vi "VHist - Time Range from history array.vi"(1 "history array":T1(array[cluster]) {"history data" format="%.2f"; "time stamps" format="%<%H:%M:%S%2u\n%d/%m/%Y>T"}) -> (4 "max time stamp":dbl format="%<%H:%M:%S%2u\n%d/%m/%Y>T", 5 "min time stamp":dbl format="%<%H:%M:%S%2u\n%d/%m/%Y>T")   [LabVIEW 2021]
doc: "The VI looks over several DBL histories and returns the oldest and the newest time stamps found.\n\n::: CalcExpress Toolkit :::\nCopyright (c) 2000-2026 Konstantin Shifershteyn. All rights reserved."
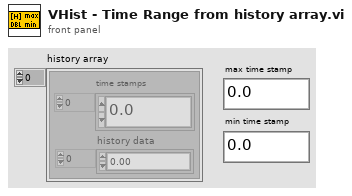
[diagram p1: front panel]
types:
  T1 = cluster{"time stamps":dbl[], "history data":dbl[]}[]
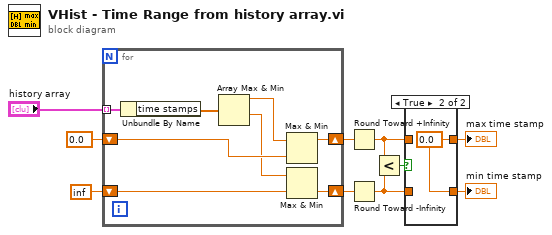
[diagram p0: block diagram]
diagram:
  n1 = for {
    tunnel: "history array" -> [w17] mode=indexing
    shift-right: [w16] -> w5
    shift-left: 0.0 -> [w15]
    shift-right: [w13] -> w4
    shift-left: inf -> [w11]
    n2 = Unbundle By Name(w17) -> ("time stamps"=w18:dbl[])
    n3 = Array Max & Min(array=w18) -> (max value=w14:dbl, min value=w12:dbl)  [unwired: 2 out]
    n4 = Max & Min(x=w14, y=w15) -> (max(x,y)=w16:dbl)  [unwired: 1 out]
    n5 = Max & Min(x=w12, y=w11) -> (min(x,y)=w13:dbl)  [unwired: 1 out]
  }
  n6 = Round Toward +Infinity(x=w5) -> (ceil(x): smallest int >= x=w1:dbl)
  n7 = Round Toward -Infinity(1:w4) -> (0:w2:dbl)
  n8 = Less?(x=w1, y=w2) -> (x < y?=w3:bool)
  n9 = case shown="True" w3 {
    tunnel: w2 -> [w19 _]
    tunnel: w1 -> [w20 _]
    tunnel: [w20 w21] -> w9
    tunnel: [w19 w21] -> w8
    frame False {
    }
    frame True {
      w21 = 0.0
    }
  }
  "min time stamp" <- w8
  "max time stamp" <- w9
